vi "Housekeeping.vi"(8 "error in (no error)":errorcluster, 11 "CIFPlugin in":refnum<class "CAN_Reader_CANsub_Plugin.lvclass">) -> (0 "error out":errorcluster, 3 "CIFPlugin out":refnum<class "CAN_Reader_CANsub_Plugin.lvclass">)   [LabVIEW 2021, in "CAN_Reader_CANsub_Plugin.lvclass"]
uses:
  CAN_Reader_CANsub_Plugin.lvclass
  CAN_Reader_CANsub_Plugin.lvclass/CAN_Reader_CANsub_Plugin.ctl
  <vilib>/CIF Foundation/CIF Core/CIFCore/Class/CIFCorePlugin.lvclass
  <vilib>/CIF Foundation/CIF Core/CIFCore/Class/Typedef/Energized States.ctl
  C:/Program Files/National Instruments/LabVIEW 2021/vi.lib/CIF Foundation/CIF Core/CIFCore/Class/CIFCorePlugin.lvclass
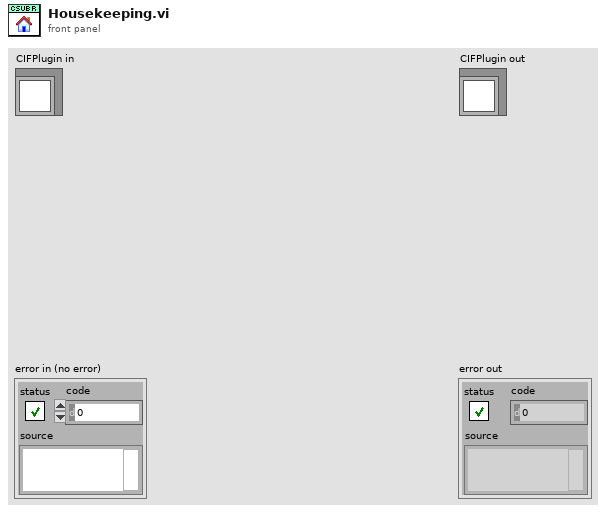
[diagram p1: front panel]
types:
  T1 = typedef "CIFCorePlugin.lvclass/Energized States.ctl" = enum8{"Listen", "Prepare", "Execute", "Housekeep", "Cleanup", "Destroy"}
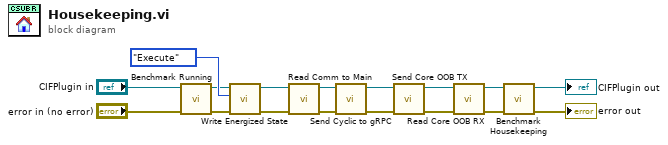
[diagram p0: block diagram]
diagram:
  n1 = call <vilib>:"Benchmark Running.vi"("error in (no error)"="error in (no error)", "CIFCorePlugin in"="CIFPlugin in") -> ("error out"=w13:errorcluster, "CIFCorePlugin out"=w8:refnum<class "CAN_Reader_CANsub_Plugin.lvclass">)  [unwired: 8 in]
  n2 = call <vilib>:"Write Energized State.vi"("error in (no error)"=w13, "Energized State"=Energized_States."Execute", "CIFCorePlugin in"=w8) -> ("error out"=w12:errorcluster, "CIFCorePlugin out"=w10:refnum<class "CAN_Reader_CANsub_Plugin.lvclass">)  [unwired: 7 in]
  n3 = call "Read Comm to Main.vi"("error in (no error)"=w12, "CIFPlugin in"=w10) -> ("error out"=w14:errorcluster, "CIFPlugin out"=w15:refnum<class "CAN_Reader_CANsub_Plugin.lvclass">)  [unwired: 8 in]
  n4 = call "Send Cyclic to gRPC.vi"("error in (no error)"=w14, "CIFPlugin in"=w15) -> ("error out"=w16:errorcluster, "CIFPlugin out"=w11:refnum<class "CAN_Reader_CANsub_Plugin.lvclass">)  [unwired: 8 in]
  n5 = call <vilib>:"Send Core OOB TX.vi"("error in (no error)"=w16, "CIFCorePlugin in"=w11) -> ("error out"=w17:errorcluster, "CIFCorePlugin out"=w7:refnum<class "CAN_Reader_CANsub_Plugin.lvclass">)  [unwired: 8 in]
  n6 = call <vilib>:"Read Core OOB RX.vi"("error in (no error)"=w17, "CIFCorePlugin in"=w7) -> ("error out"=w3:errorcluster, "CIFCorePlugin out"=w4:refnum<class "CAN_Reader_CANsub_Plugin.lvclass">)  [unwired: 8 in]
  n7 = call <vilib>:"Benchmark Housekeeping.vi"("error in (no error)"=w3, "CIFCorePlugin in"=w4) -> ("error out"=→"error out":errorcluster, "CIFCorePlugin out"=→"CIFPlugin out":refnum<class "CAN_Reader_CANsub_Plugin.lvclass">)  [unwired: 8 in]
